vi "Initialise.vi"(5 "End row Cell position:":cluster{"row":i32, "column":i32}={"row"=3, "column"=3}, 7 "Start row Cell position:":cluster{"row":i32, "column":i32}={"row"=3, "column"=1}, 8 "Excel template path":path, 9 "Source X":refnum<visa-resource-name>, 10 "Source Ref":refnum<visa-resource-name>, 11 "Voltmeter":refnum<visa-resource-name>) -> (0 "references":T1, 1 "end row":i32, 2 "start row":i32, 3 "measurement settings":string[][](array[string]))   [LabVIEW 2011]
doc: "Initialise instruments and loads measurement data from excel template."
uses:
  Measurement References.ctl
  <vilib>/Utility/NIReport.llb/NI_report.lvclass
  <vilib>/addons/_office/excel.llb/Excel Get Data (i32).vi
  <vilib>/addons/_office/excel.llb/Excel Get Data ([str]).vi
  <vilib>/Utility/NIReport.llb/Excel/NI_Excel.lvclass
  <vilib>/addons/_office/NI_ReportGenerationToolkit.lvlib
  <instrlib>/Fluke 5XXX Series Multicalibrators/Fluke 5XXX Series Multicalibrators.lvlib
panel:
  in  "references constant":T1
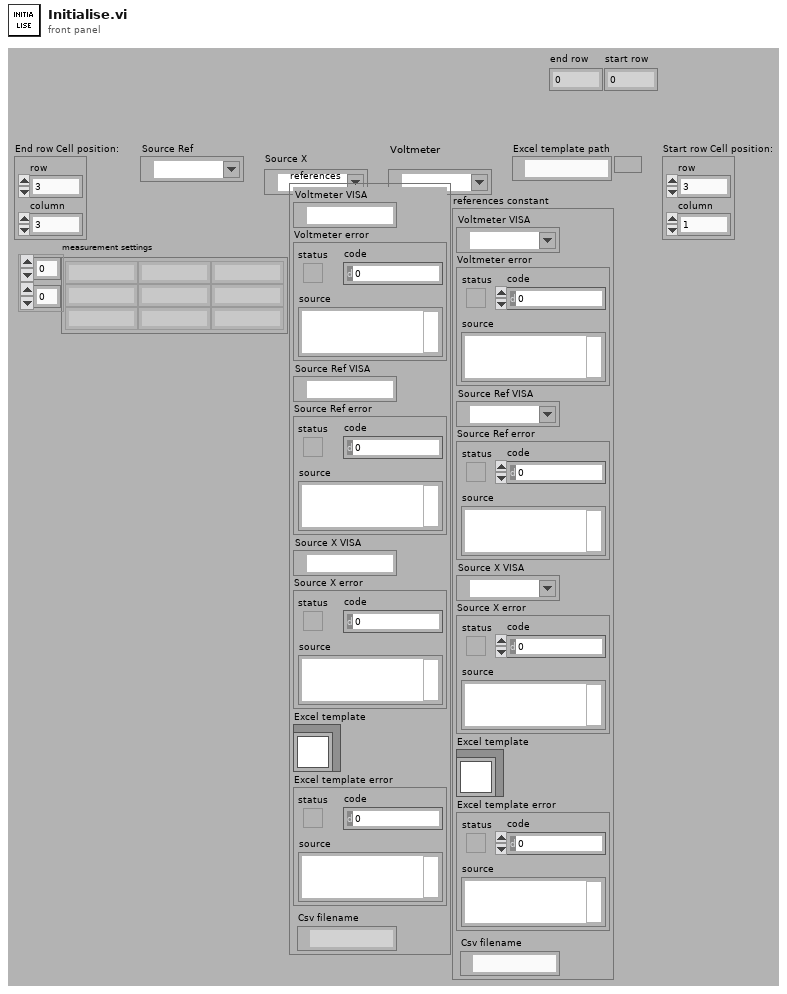
[diagram p1: front panel]
types:
  T1 = typedef "Measurement References.ctl" = cluster{"Voltmeter VISA":refnum<visa-resource-name>, "Voltmeter error":errorcluster, "Source Ref VISA":refnum<visa-resource-name>, "Source Ref error":errorcluster, "Source X VISA":refnum<visa-resource-name>, "Source X error":errorcluster, "Excel template":refnum<class "NI_report.lvclass">, "Excel template error":errorcluster, "Csv filename":path}
  T2 = enum16{"Standard Report", "HTML", "Word", "Excel"}
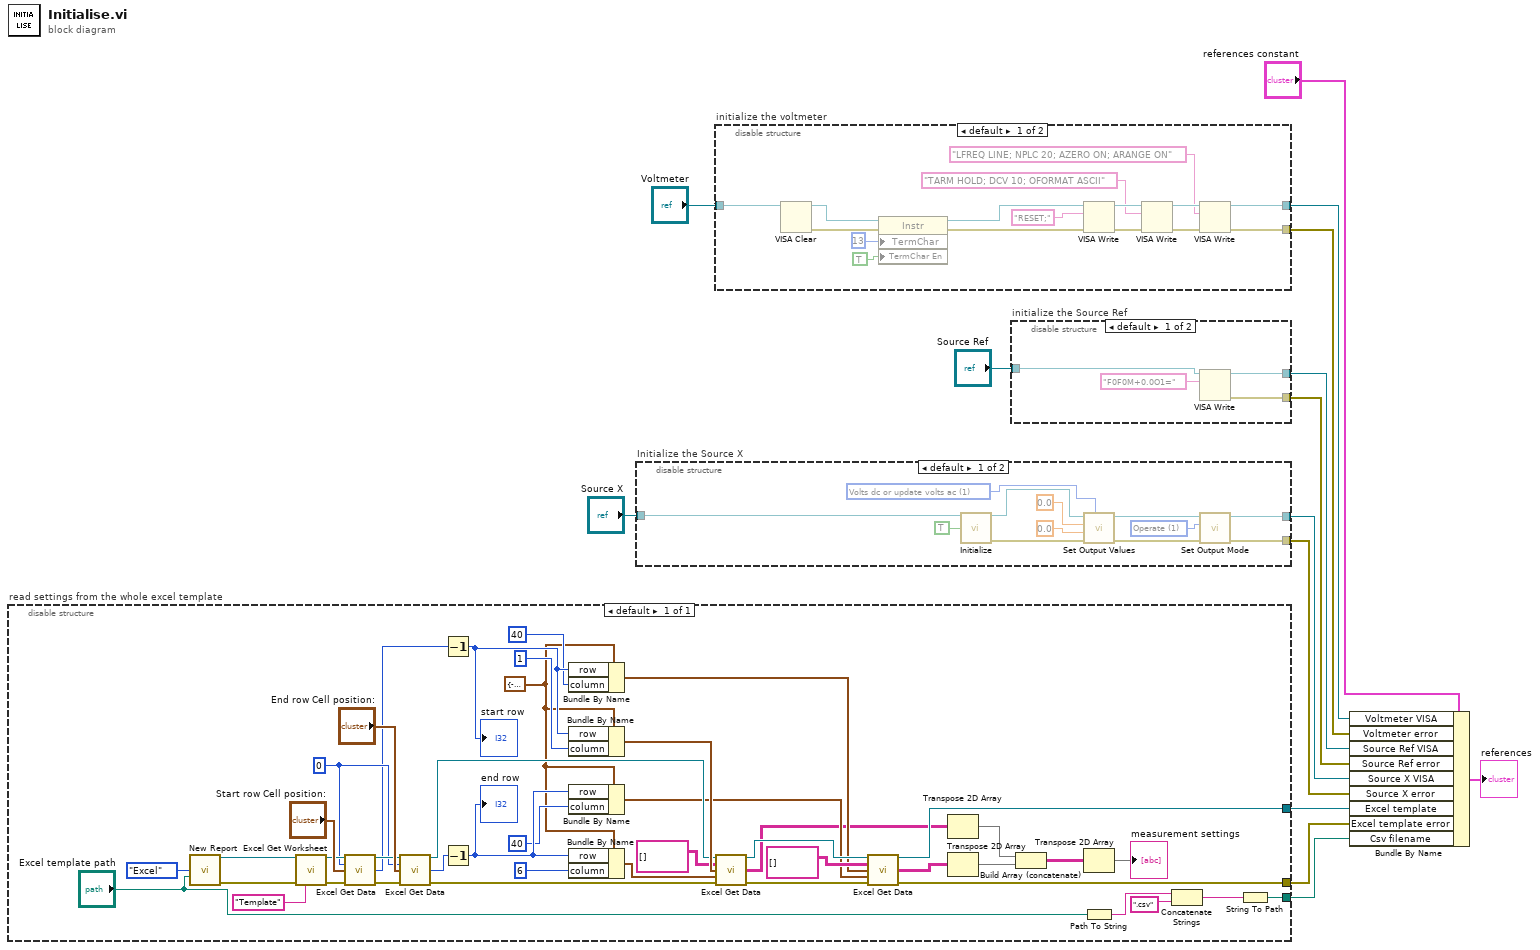
[diagram p0: block diagram]
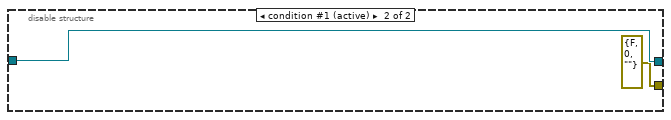
[diagram p2: hidden frame]
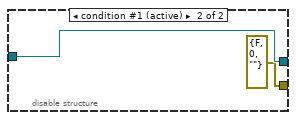
[diagram p3: hidden frame]
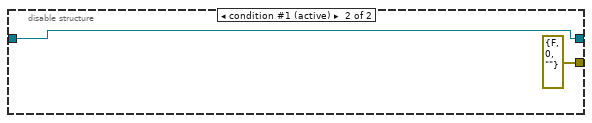
[diagram p4: hidden frame]
diagram:
  n1 = disable-structure "read settings from the whole excel template" shown="default" {
    disable-tunnel: [w34] -> w4
    disable-tunnel: [w33] -> w3
    disable-tunnel: [w15] -> w1
    frame Enabled {
      w27 = cluster{"row":i32, "column":i32} {"row"=-1, "column"=-1} ("End row Cell position:")
      w47 = 0
      n2 = call <vilib>:"New Report.vi"("report type"=T2."Excel", "template (empty)"="Excel template path") -> ("report out"=w49:refnum<class "NI_report.lvclass">, "error out"=w50:errorcluster)  [unwired: 12 in]
      n3 = call <vilib>:"Excel Get Worksheet.vi"("report in"=w49, "error in (no error)"=w50, "name (\"\")"="Template" ("name (\"\")")) -> ("report out"=w52:refnum<class "NI_report.lvclass">, "error out"=w53:errorcluster)  [unwired: 11 in]
      n4 = call-poly <vilib>:"Excel Get Data.vi"("report in"=w52, "data type"=w47, "start (0, 0)"="Start row Cell position:", "error in (no error)"=w53) -> ("report out"=w55:refnum<class "NI_report.lvclass">, "data"=w39:i32, "error out"=w56:errorcluster)  [unwired: 9 in]
      n5 = call-poly <vilib>:"Excel Get Data.vi"("report in"=w55, "data type"=w47, "start (0, 0)"="End row Cell position:", "error in (no error)"=w56) -> ("report out"=w41:refnum<class "NI_report.lvclass">, "data"=w38:i32, "error out"=w40:errorcluster)  [unwired: 9 in]
      n6 = Decrement(x=w39) -> (x-1=w31:i32)
      "start row" <- w31
      n7 = Decrement(x=w38) -> (x-1=w32:i32)
      "end row" <- w32
      n8 = Bundle By Name(cluster=w27, "row"=w31, "column"=40) -> (w28:cluster{"row":i32, "column":i32})
      n9 = Bundle By Name(cluster=w27, "row"=w31, "column"=1) -> (w46:cluster{"row":i32, "column":i32})
      n10 = Bundle By Name(cluster=w27, "row"=w32, "column"=40) -> (w26:cluster{"row":i32, "column":i32})
      n11 = Bundle By Name(cluster=w27, "row"=w32, "column"=6) -> (w43:cluster{"row":i32, "column":i32})
      n12 = call-poly <vilib>:"Excel Get Data.vi"("report in"=w41, "data type"=string[][] [], "start (-1, -1)"=w46, "end (-1, -1)"=w43, "error in (no error)"=w40) -> ("report out"=w36:refnum<class "NI_report.lvclass">, "data"=w25:string[][], "error out"=w35:errorcluster)  [unwired: 8 in]
      n13 = call-poly <vilib>:"Excel Get Data.vi"("report in"=w36, "data type"=string[][] [], "start (-1, -1)"=w28, "end (-1, -1)"=w26, "error in (no error)"=w35) -> ("report out"=w34:refnum<class "NI_report.lvclass">, "data"=w23:string[][], "error out"=w33:errorcluster)  [unwired: 8 in]
      n14 = Transpose 2D Array(2D array=w25) -> (transposed array=w24:string[][])
      n15 = Transpose 2D Array(2D array=w23) -> (transposed array=w22:string[][])
      n16 = Build Array (concatenate)(w24, w22) -> (w21:string[][])
      n17 = Transpose 2D Array(2D array=w21) -> (transposed array=→"measurement settings":string[][])
      n18 = Path To String(path="Excel template path") -> (string=w19:string)
      n19 = Concatenate Strings(w19, ".csv" ("string")) -> (w18:string)
      n20 = String To Path(string=w18) -> (path=w15:path)
    }
  }
  n21 = disable-structure "Initialize the Source X" shown="default" {
    disable-tunnel: "Source X" -> [w61 w71]
    disable-tunnel: [w59 w71] -> w10
    disable-tunnel: [w58 errorcluster {"status"=FALSE, "code"=0, "source"=""} ("error out")] -> w9
    frame condition #0 {
      w67 = u32 1 items=["Amplitude", "Volts dc or update volts ac", "Volts ac dBm update", "Volts ac or volts dc with 0 Hz", "Volts ac in dBm", "Current dc or update current ac", "Current ac", "Update frequency", "Resistance", "Capacitance", "Temperature (Celsius)", "Temperature (Fahrenheit)", "Power dc or update power ac", "Power ac", "Dual volts dc or update dual ac", "Dual volts ac in volts", "Power ac in dBm update", "Power ac in dBm", "Dual volts ac in dBm update", "Dual volts ac in dBm"] ("Output Value(s) (0 - Amplitude)")
      w66 = u32 1 items=["Standby", "Operate"] ("Output Mode (0: Standby)")
      n22 = call <instrlib>:"Initialize.vi"("VISA resource name"=w61, "Reset (T: Reset)"=TRUE) -> ("VISA resource name out"=w62:refnum<visa-resource-name>, "error out"=w63:errorcluster)  [unwired: 12 in]
      n23 = call <instrlib>:"Set Output Values.vi"("Output Value(s) (0 - Amplitude)"=w67, "error in (no error)"=w63, "Secondary Value (0.0)"=0.0, "Primary Value (0.0)"=0.0, "VISA resource name"=w62) -> ("error out"=w69:errorcluster, "VISA resource name out"=w68:refnum<visa-resource-name>)  [unwired: 5 in]
      n24 = call <instrlib>:"Set Output Mode.vi"("error in (no error)"=w69, "Output Mode (0: Standby)"=w66, "VISA resource name"=w68) -> ("error out"=w58:errorcluster, "VISA resource name out"=w59:refnum<visa-resource-name>)  [unwired: 7 in]
    }
    frame condition #1 (active) {
    }
  }
  n25 = disable-structure "initialize the voltmeter" shown="default" {
    disable-tunnel: "Voltmeter" -> [w87 w89]
    disable-tunnel: [w86 w89] -> w8
    disable-tunnel: [w85 errorcluster {"status"=FALSE, "code"=0, "source"=""} ("error out")] -> w7
    frame condition #0 {
      n26 = VISA Clear(VISA resource name=w87) -> (VISA resource name out=w75:refnum<visa-resource-name>, error out=w74:errorcluster)  [unwired: 1 in]
      n27 = property class="Instr"(reference=w75, error in=w74, "TermChar"=u8 13 ("Message Based Settings:Termination Character"), "TermChar En"=TRUE ("Message Based Settings:Termination Character Enable")) -> (reference out=w73:refnum<visa-resource-name>, error out=w72:errorcluster)
      n28 = VISA Write(VISA resource name=w73, write buffer="RESET;", error in (no error)=w72) -> (VISA resource name out=w81:refnum<visa-resource-name>, error out=w80:errorcluster)  [unwired: 1 out]
      n29 = VISA Write(VISA resource name=w81, write buffer="TARM HOLD; DCV 10; OFORMAT ASCII", error in (no error)=w80) -> (VISA resource name out=w82:refnum<visa-resource-name>, error out=w83:errorcluster)  [unwired: 1 out]
      n30 = VISA Write(VISA resource name=w82, write buffer="LFREQ LINE; NPLC 20; AZERO ON; ARANGE ON", error in (no error)=w83) -> (VISA resource name out=w86:refnum<visa-resource-name>, error out=w85:errorcluster)  [unwired: 1 out]
    }
    frame condition #1 (active) {
    }
  }
  n31 = disable-structure "initialize the Source Ref" shown="default" {
    disable-tunnel: "Source Ref" -> [w92 w95]
    disable-tunnel: [w91 w95] -> w12
    disable-tunnel: [w90 errorcluster {"status"=FALSE, "code"=0, "source"=""} ("error out")] -> w11
    frame condition #0 {
      n32 = VISA Write(VISA resource name=w92, write buffer="F0F0M+0.0O1=") -> (VISA resource name out=w91:refnum<visa-resource-name>, error out=w90:errorcluster)  [unwired: 1 in, 1 out]
    }
    frame condition #1 (active) {
    }
  }
  n33 = Bundle By Name(cluster="references constant", "Voltmeter VISA"=w8, "Voltmeter error"=w7, "Source Ref VISA"=w12, "Source Ref error"=w11, "Source X VISA"=w10, "Source X error"=w9, "Excel template"=w4, "Excel template error"=w3, "Csv filename"=w1) -> (→"references":T1)
